vi "Write Address.vi"(8 "error in (no error)":errorcluster, 10 "address":string, 11 "Modbus_TCP in":refnum<class "Modbus_TCP.lvclass">) -> (0 "error out":errorcluster, 3 "Modbus_TCP out":refnum<class "Modbus_TCP.lvclass">)   [LabVIEW 2021, in "Modbus_TCP.lvclass"]
uses:
  Modbus_TCP.lvclass
  Modbus_TCP.lvclass/Modbus_TCP.ctl
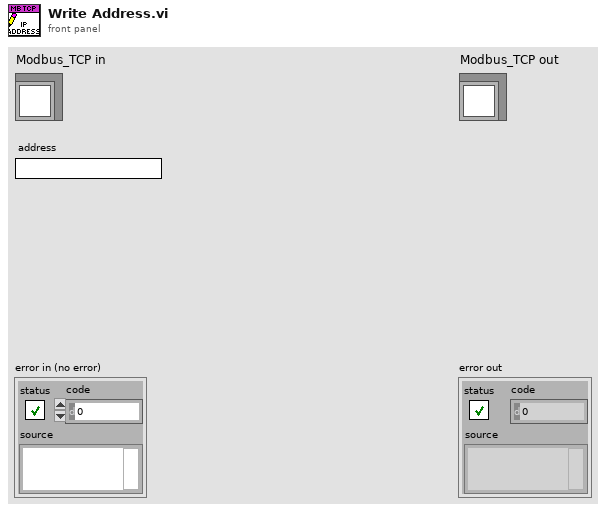
[diagram p1: front panel]
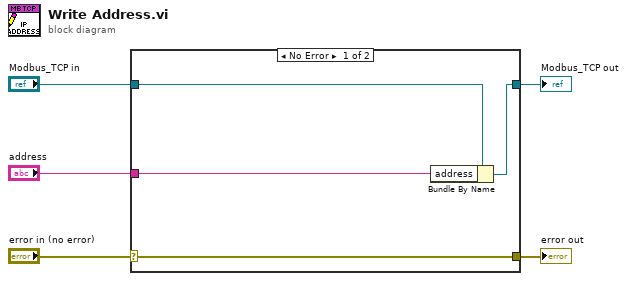
[diagram p0: block diagram]
diagram:
  n1 = case shown="No Error" "error in (no error)" {
    selector: "error in (no error)" -> [w9 w10]
    tunnel: [w9 w10] -> w4
    tunnel: [w7 w11] -> w2
    tunnel: "Modbus_TCP in" -> [w8 w11]
    tunnel: "address" -> [w6 _]
    frame No Error {
      n2 = Bundle By Name(cluster=w8, "address"=w6) -> (w7:refnum<class "Modbus_TCP.lvclass">)
    }
    frame Error {
    }
  }
  "error out" <- w4
  "Modbus_TCP out" <- w2
